vi "Finish Stream.vi"(8 "error in":errorcluster, 9 "response":string, 10 "cancelled":refnum<queue>, 11 "events":refnum<queue>) -> (0 "error out":errorcluster)   [LabVIEW 2020, in "MCP Server.lvlib"]
doc: "Ends a streamed tools/call. When response is not empty it is sent as the last event \"data: <response>\" (line breaks removed, so it stays one SSE data line); then the end marker (an empty string) is put on the events queue, which makes the MCP SSE Response close the stream. Waits at most 5 s for the stream to take the events and releases both queues of the MCP SSE Response.\n\nRuns regardless of error in. error out is error in merged with the errors of the queue operations."
uses:
  MCP Server.lvlib
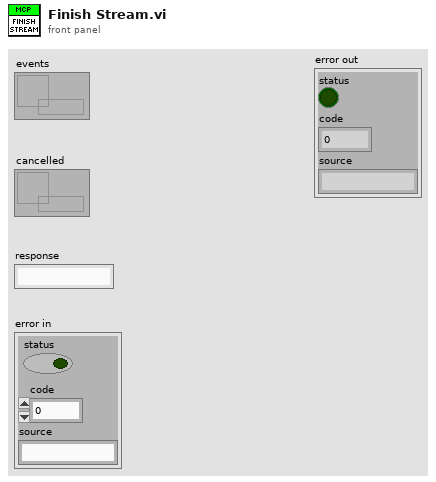
[diagram p1: front panel]
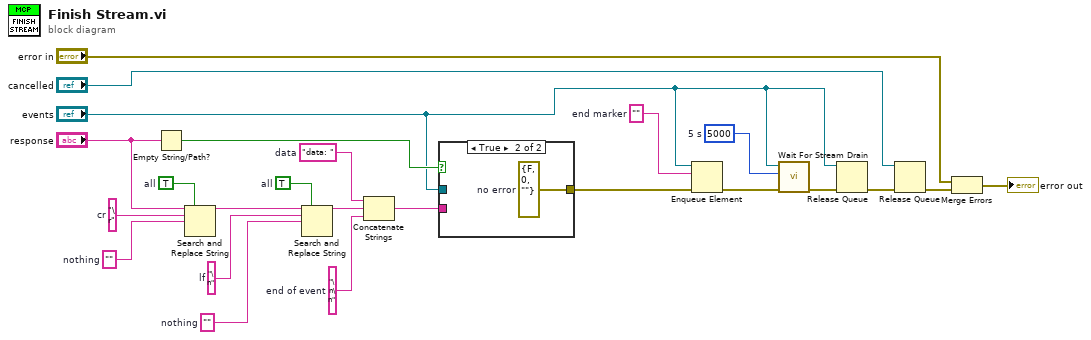
[diagram p0: block diagram]
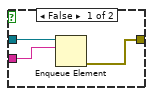
[diagram p2: hidden frame]
diagram:
  w14 = 5000  # 5 s
  w13 = ""  # end marker
  w12 = "\n\n"  # end of event
  w11 = "data: "  # data
  w10 = TRUE  # all
  w9 = TRUE  # all
  w8 = ""  # nothing
  w7 = ""  # nothing
  w6 = "\n"  # lf
  w5 = "\r"  # cr
  n1 = Empty String/Path?(string/path="response") -> (empty?=w15:bool)
  n2 = Search and Replace String(replace all?=w9, input string="response", search string=w5, replace string=w7) -> (result string=w16:string)  [unwired: 4 in, 3 out]
  n3 = Search and Replace String(replace all?=w10, input string=w16, search string=w6, replace string=w8) -> (result string=w17:string)  [unwired: 4 in, 3 out]
  n4 = Concatenate Strings(w11, w17, w12) -> (w18:string)
  n5 = case shown="True" w15 {
    tunnel: "events" -> [w25 _]
    tunnel: w18 -> [w26 _]
    tunnel: [w27 w28] -> w19
    frame False {
      n6 = Enqueue Element(queue=w25, element=w26) -> (error out=w27:errorcluster)  [unwired: 2 in, 2 out]
    }
    frame True {
      w28 = errorcluster {"status"=FALSE, "code"=0, "source"=""}  # no error
    }
  }
  n7 = Enqueue Element(queue="events", element=w13, error in (no error)=w19) -> (error out=w20:errorcluster)  [unwired: 1 in, 2 out]
  n8 = call "Wait For Stream Drain.vi"("error in"=w20, "timeout ms"=w14, "events"="events") -> ("error out"=w21:errorcluster)  [unwired: 7 in, 1 out]
  n9 = Release Queue(queue="events", error in (no error)=w21) -> (error out=w22:errorcluster)  [unwired: 1 in, 2 out]
  n10 = Release Queue(queue="cancelled", error in (no error)=w22) -> (error out=w23:errorcluster)  [unwired: 1 in, 2 out]
  n11 = Merge Errors("error in", w23) -> (→"error out":errorcluster)
